vi "Exit with Code.vi"(8 "error in (no error)":errorcluster, 10 "Exit Code (0)":i32, 11 "CLI in":refnum<class "CLI.lvclass">) -> (0 "error out":errorcluster)   [LabVIEW 2015, in "CLI.lvclass"]
doc: "Ends the command line executable with the exit code provided.\n\nCall this when your application ends to ensure the caller see's that it has ended."
uses:
  CLI.lvclass
  CLI.lvclass/CLI.ctl
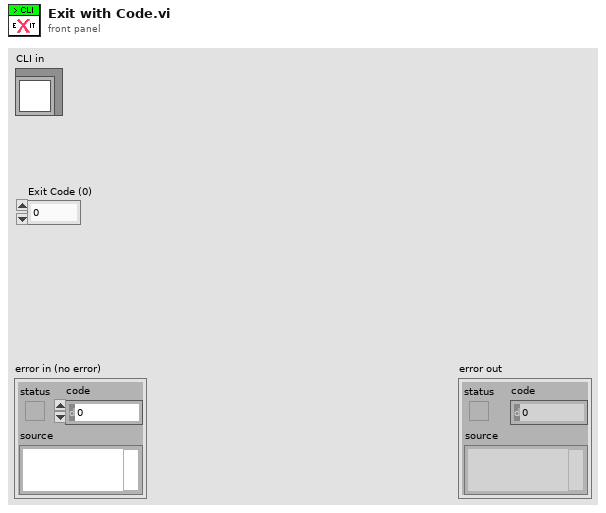
[diagram p1: front panel]
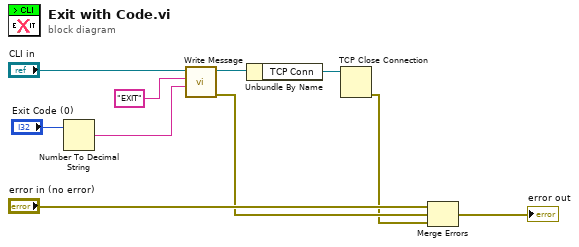
[diagram p0: block diagram]
diagram:
  n1 = Number To Decimal String(number="Exit Code (0)") -> (decimal integer string=w1:string)  [unwired: 1 in]
  n2 = call "Write Message.vi"("Message Contents"=w1, "Message Type"="EXIT", "CLI in"="CLI in") -> ("error out"=w3:errorcluster, "CLI out"=w6:refnum<class "CLI.lvclass">)  [unwired: 7 in]
  n3 = Unbundle By Name(w6) -> ("TCP Conn"=w5:refnum<k5>)
  n4 = TCP Close Connection(connection ID=w5) -> (error out=w2:errorcluster)  [unwired: 2 in, 1 out]
  n5 = Merge Errors("error in (no error)", w3, w2) -> (→"error out":errorcluster)
